vi "Start Story.vi"(11 "market":T1) -> (3 "market out":T1)   [LabVIEW 2020, in "Full Featured MCP Server.lvlib"]
doc: "Now and then starts a new story from the Story Catalogue: picks a story that is not running yet, casts a lead stock (from the leads of the story, or any stock) and a second stock, and schedules the first step. At most 3 stories run at once."
uses:
  Full Featured MCP Server.lvlib
  Market State.ctl
  News Item.ctl
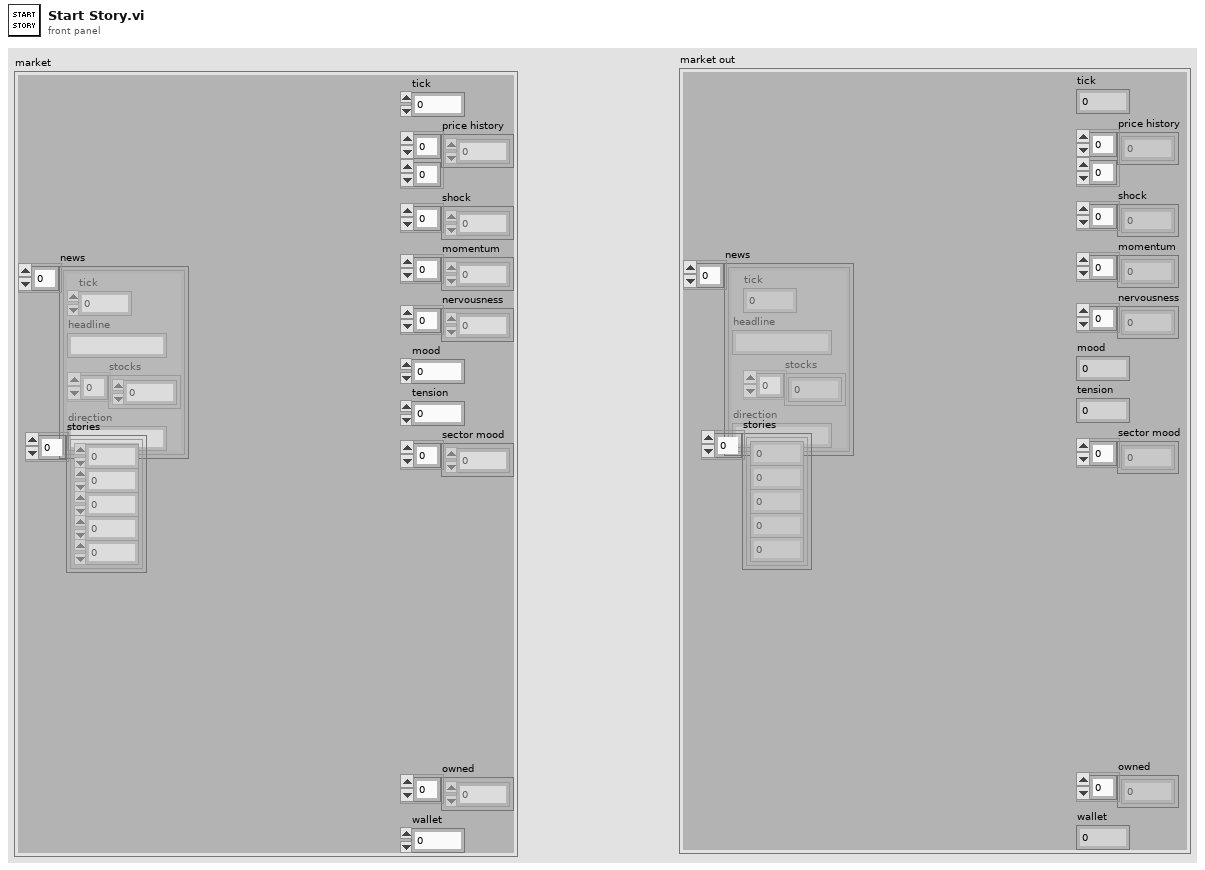
[diagram p1: front panel]
types:
  T1 = typedef "Full Featured MCP Server.lvlib/Market State.ctl" = cluster{"tick":i32, "price history":dbl[][], "shock":dbl[], "momentum":dbl[], "nervousness":dbl[], "mood":dbl, "tension":dbl, "sector mood":dbl[], "news":T2[], "stories":cluster{"arc":i32, "step":i32, "due":i32, "stock":i32, "other":i32}[], "owned":i32[], "wallet":dbl}
  T2 = typedef "Full Featured MCP Server.lvlib/News Item.ctl" = cluster{"tick":i32, "headline":string, "stocks":i32[], "direction":string}
  T3 = cluster{"title":string, "first step":i32, "leads":i32[]}[]
  T4 = cluster{"arc":i32, "step":i32, "due":i32, "stock":i32, "other":i32}[]
  T5 = cluster{"arc":i32, "step":i32, "due":i32, "stock":i32, "other":i32}
  T6 = cluster{"title":string, "first step":i32, "leads":i32[]}
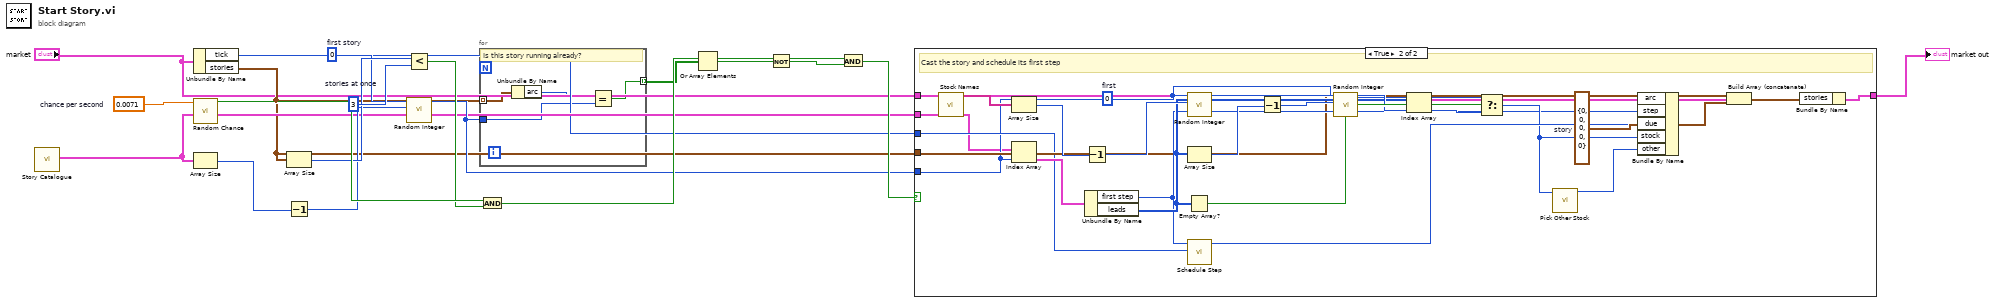
[diagram p0: block diagram]
diagram:
  w14 = 0.0071  # chance per second
  w12 = 3  # stories at once
  w5 = 0  # first story
  n1 = call "Story Catalogue.vi"() -> ("arcs"=w4:T3)  [unwired: 10 in, 1 out]
  n2 = Unbundle By Name("market") -> ("tick"=w2:i32, "stories"=w3:T4)
  n3 = call "Random Chance.vi"("probability"=w14) -> ("happened?"=w15:bool)  [unwired: 10 in]
  n4 = Array Size(array=w4) -> (size(s)=w6:i32)
  n5 = Array Size(array=w3) -> (size(s)=w11:i32)
  n6 = Decrement(x=w6) -> (x-1=w7:i32)
  n7 = Less?(x=w11, y=w12) -> (x < y?=w13:bool)
  n8 = call "Random Integer.vi"("high"=w7, "low"=w5) -> ("number"=w8:i32)  [unwired: 9 in]
  n9 = for {
    tunnel: w3 -> [w20] mode=indexing
    tunnel: w8 -> [w22]
    tunnel: [w23] -> w9 mode=indexing
    # "Is this story running already?"
    n10 = Unbundle By Name(w20) -> ("arc"=w21:i32)
    n11 = Equal?(x=w21, y=w22) -> (x = y?=w23:bool)
  }
  n12 = And(x=w15, y=w13) -> (x .and. y?=w16:bool)
  n13 = Or Array Elements(Boolean array=w9) -> (logical OR=w10:bool)
  n14 = Not(x=w10) -> (.not. x?=w17:bool)
  n15 = And(x=w16, y=w17) -> (x .and. y?=w18:bool)
  n16 = case shown="True" w18 {
    tunnel: "market" -> [w24 w29]
    tunnel: w4 -> [_ w25]
    tunnel: w2 -> [_ w27]
    tunnel: w3 -> [_ w28]
    tunnel: w8 -> [_ w26]
    tunnel: [w24 w30] -> w19
    frame False {
      # "No new story"
    }
    frame True {
      w47 = T5 {"arc"=0, "step"=0, "due"=0, "stock"=0, "other"=0}  # story
      w36 = 0  # first
      # "Cast the story and schedule its first step"
      n17 = call "Stock Names.vi"() -> ("names"=w34:string[])  [unwired: 11 in]
      n18 = Array Size(array=w34) -> (size(s)=w35:i32)
      n19 = Index Array(array=w25, index=w26) -> (element=w31:T6)
      n20 = Decrement(x=w35) -> (x-1=w37:i32)
      n21 = Unbundle By Name(w31) -> ("first step"=w32:i32, "leads"=w33:i32[])
      n22 = call "Random Integer.vi"("high"=w37, "low"=w36) -> ("number"=w38:i32)  [unwired: 9 in]
      n23 = Array Size(array=w33) -> (size(s)=w39:i32)
      n24 = Empty Array?(array=w33) -> (empty?=w43:bool)
      n25 = call "Schedule Step.vi"("now"=w27, "step"=w32) -> ("due"=w46:i32)  [unwired: 9 in]
      n26 = Decrement(x=w39) -> (x-1=w40:i32)
      n27 = call "Random Integer.vi"("high"=w40, "low"=w36) -> ("number"=w41:i32)  [unwired: 9 in]
      n28 = Index Array(array=w33, index=w41) -> (element=w42:i32)
      n29 = Select(t=w38, s=w43, f=w42) -> (s? t:f=w44:i32)
      n30 = call "Pick Other Stock.vi"("stock"=w44) -> ("other"=w45:i32)  [unwired: 10 in]
      n31 = Bundle By Name(cluster=w47, "arc"=w26, "step"=w32, "due"=w46, "stock"=w44, "other"=w45) -> (w48:T5)
      n32 = Build Array (concatenate)(w28, w48) -> (w49:T4)
      n33 = Bundle By Name(cluster=w29, "stories"=w49) -> (w30:T1)
    }
  }
  "market out" <- w19
